vi "RT Loop - Publish IO.vi"() -> ()   [LabVIEW 2018]
uses:
  <vilib>/Skyline/Tag/Shared/typedefs/DataType.ctl
  <vilib>/Skyline/Tag/Shared/typedefs/Retention Type.ctl
  <vilib>/Skyline/Configuration/Configuration AMQP_class/Open Configuration AMQP.vi
  <vilib>/Skyline/Tag/Wrapper/Wrapper AMQP_class/Open Tag AMQP.vi
  <vilib>/Skyline/Tag/Wrapper/Wrapper_class/Generate Tag Cluster (DBL) 2.vi
  <vilib>/Skyline/Tag/Wrapper/Wrapper_class/NI Skyline Tag.lvclass
  <vilib>/Skyline/Configuration/Configuration_class/NI Skyline Configuration.lvclass
  <vilib>/Skyline/Configuration/Configuration HTTP_class/NI Skyline Configuration HTTP.lvclass
  <vilib>/Skyline/Configuration/Configuration AMQP_class/NI Skyline Configuration AMQP.lvclass
  <vilib>/Skyline/Tag/Shared/NI Skyline Tag.lvlib
  <vilib>/Skyline/Tag/Wrapper/Wrapper AMQP_class/NI Skyline Tag AMQP.lvclass
panel:
  out "error out":errorcluster
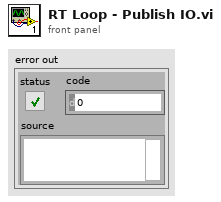
[diagram p1: front panel]
types:
  T1 = typedef "NI Skyline Tag.lvlib/Retention Type.ctl" = enum32{"None", "Duration", "Count", "Permanent"}
  T2 = typedef "NI Skyline Tag.lvlib/DataType.ctl" = enum32{"Double", "I32", "String", "Boolean", "U64", "Timestamp"}
  T3 = typedef "NI Skyline Tag.lvclass/Tag Value Cluster Wrapper.ctl" = cluster{"Configuration":refnum<class "NI Skyline Configuration.lvclass">, "Tag Cluster":T4}
  T4 = typedef "NI Skyline Tag.lvlib/Tag Value Cluster.ctl" = cluster{"Path":string, "Data Type":T2, "Value":string, "Time Stamp":timestamp}
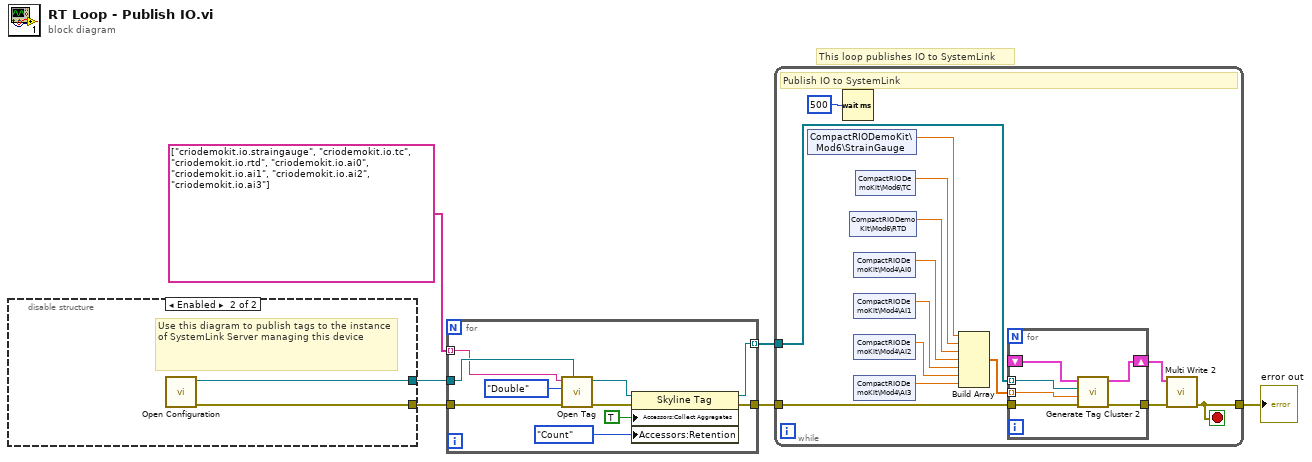
[diagram p0: block diagram]
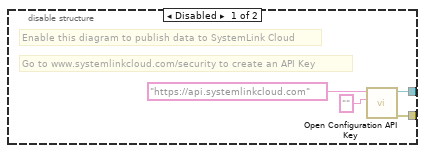
[diagram p2: hidden frame]
diagram:
  # "This loop publishes IO to SystemLink"
  n1 = disable-structure shown="Enabled" {
    disable-tunnel: [w8 w12] -> w6
    disable-tunnel: [w7 w11] -> w4
    frame Disabled {
      # "Enable this diagram to publish data to SystemLink Cloud"
      # "Go to www.systemlinkcloud.com/security to create an API Key"
      n2 = call <vilib>:"Open Configuration API Key.vi"("api key"="", "server url"="https://api.systemlinkcloud.com") -> ("error out"=w7:errorcluster, "HTTP configuration out"=w8:refnum<class "NI Skyline Configuration HTTP.lvclass">)  [unwired: 8 in]
    }
    frame Enabled {
      # "Use this diagram to publish tags to the instance of SystemLink Server managing this device"
      n3 = call-poly <vilib>:"Open Configuration.vi"() -> ("error out"=w11:errorcluster, "AMQP configuration out"=w12:refnum<class "NI Skyline Configuration AMQP.lvclass">)  [unwired: 10 in]
    }
  }
  n4 = for {
    tunnel: w6 -> [w22]
    tunnel: string[] ["criodemokit.io.straingauge", "criodemokit.io.tc", "criodemokit.io.rtd", "criodemokit.io.ai0", "criodemokit.io.ai1", "criodemokit.io.ai2", "criodemokit.io.ai3"] -> [w20] mode=indexing
    tunnel: w4 -> [w19]
    tunnel: [w17] -> w3
    tunnel: [w18] -> w2 mode=indexing
    n5 = call-poly <vilib>:"Open Tag.vi"("configuration"=w22, "error in (no error)"=w19, "data type"=DataType."Double", "path"=w20) -> ("error out"=w15:errorcluster, "tag out"=w16:refnum<class "NI Skyline Tag.lvclass">)  [unwired: 6 in]
    n6 = property on="Property Node" class="Skyline Tag"(reference=w16, error in=w15, "Accessors:Collect Aggregates"=TRUE ("Collect Aggregates"), "Accessors:Retention"=Retention_Type."Count" ("Retention")) -> (reference out=w18:refnum<class "NI Skyline Tag.lvclass">, error out=w17:errorcluster)
  }
  n7 = while {
    tunnel: w3 -> [w26]
    tunnel: w2 -> [w29]
    tunnel: [w23] -> w1
    stop <- w23 stop-if-true
    # "Publish IO to SystemLink"
    n8 = shared-variable "CompactRIODemoKit\\Mod6\\StrainGauge"() -> (w36:dbl)  [unwired: 1 in, 1 out]
    n9 = Wait (ms)(milliseconds to wait=u32 500) -> ()  [unwired: 1 out]
    n10 = shared-variable "CompactRIODemoKit\\Mod6\\RTD"() -> (w34:dbl)  [unwired: 1 in, 1 out]
    n11 = shared-variable "CompactRIODemoKit\\Mod4\\AI0"() -> (w33:dbl)  [unwired: 1 in, 1 out]
    n12 = shared-variable "CompactRIODemoKit\\Mod4\\AI1"() -> (w32:dbl)  [unwired: 1 in, 1 out]
    n13 = shared-variable "CompactRIODemoKit\\Mod4\\AI2"() -> (w31:dbl)  [unwired: 1 in, 1 out]
    n14 = shared-variable "CompactRIODemoKit\\Mod4\\AI3"() -> (w30:dbl)  [unwired: 1 in, 1 out]
    n15 = shared-variable "CompactRIODemoKit\\Mod6\\TC"() -> (w35:dbl)  [unwired: 1 in, 1 out]
    n16 = Build Array(w36, w35, w34, w33, w32, w31, w30) -> (w25:dbl[])
    n17 = for {
      tunnel: w29 -> [w42] mode=indexing
      shift-right: [w41] -> w28
      shift-left: _ -> [w40]
      tunnel: [w39] -> w27
      tunnel: w26 -> [w38]
      tunnel: w25 -> [w37] mode=indexing
      n18 = call-poly <vilib>:"Generate Tag Cluster 2.vi"("error in (no error)"=w38, "value"=w37, "tag in"=w42, "tag clusters in"=w40) -> ("error out"=w39:errorcluster, "tag clusters out"=w41:T3[])  [unwired: 5 in, 1 out]
    }
    n19 = call <vilib>:"Multi Write 2.vi"("error in (no error)"=w27, "tag clusters"=w28) -> ("error out"=w23:errorcluster)  [unwired: 9 in]
  }
  "error out" <- w1
